vi "subGetBuildSpecificationRefByName.vi"(8 "error in (no error)":errorcluster, 9 "ProjectItem in":refnum<class "ProjectItem.lvclass">, 11 "BuildManager in":refnum<class "BuildManager.lvclass">) -> (0 "error out":errorcluster, 1 "Build spec ref":refnum<vi>, 3 "BuildManager out":refnum<class "BuildManager.lvclass">)   [LabVIEW 2019, in "SolutionBuilder.lvlib" / "BuildManager.lvclass"]
uses:
  BuildManager.lvclass
  ProjectItem/ProjectItem.lvclass
  ProjectItem/ProjectItem.lvclass/ProjectItem.ctl
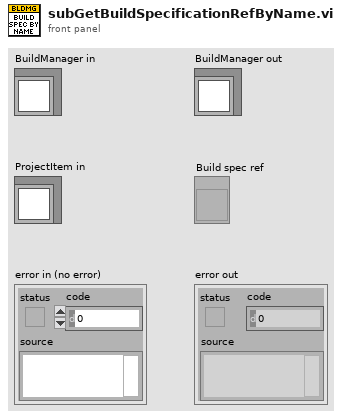
[diagram p1: front panel]
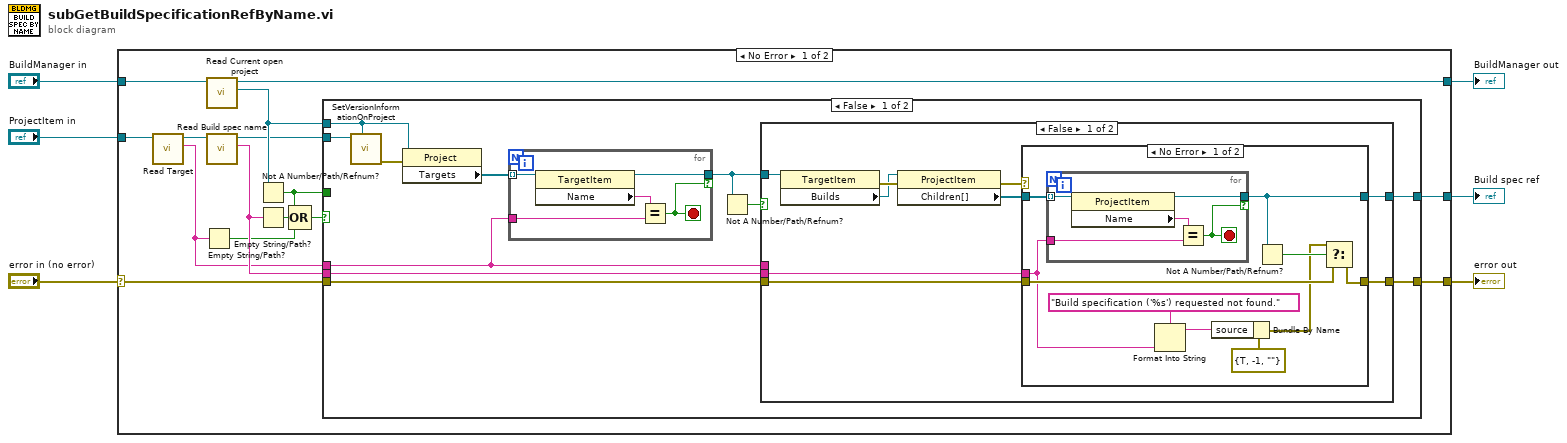
[diagram p0: block diagram]
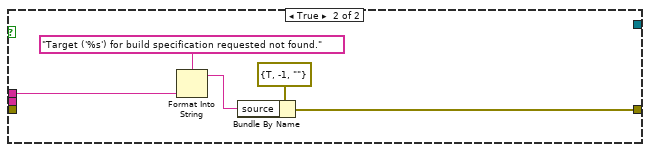
[diagram p3: hidden frame]
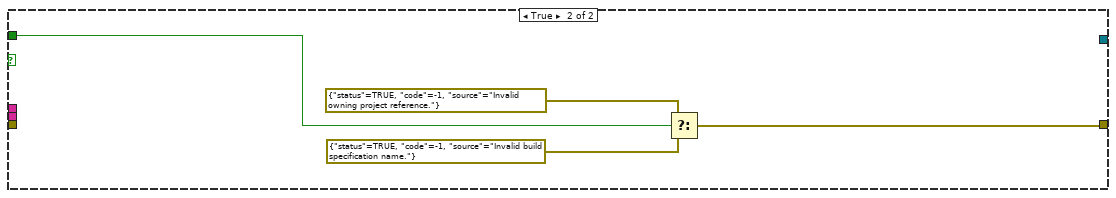
[diagram p4: hidden frame]
diagram:
  n1 = case shown="No Error" "error in (no error)" {
    selector: "error in (no error)" -> [w20 w73]
    tunnel: [w21 _] -> w6
    tunnel: [w19 w73] -> w4
    tunnel: "BuildManager in" -> [w8 w72]
    tunnel: [w15 w72] -> w2
    tunnel: "ProjectItem in" -> [w12 _]
    frame No Error {
      n2 = call "Read Target.vi"("ProjectItem in"=w12) -> ("Target"=w10:string, "ProjectItem out"=w11:refnum<class "ProjectItem.lvclass">)  [unwired: 9 in]
      n3 = Empty String/Path?(string/path=w10) -> (empty?=w9:bool)
      n4 = call "Read Current open project.vi"("BuildManager in"=w8) -> ("Current open project"=w14:refnum<vi>, "BuildManager out"=w15:refnum<class "BuildManager.lvclass">)  [unwired: 9 in]
      n5 = call "Read Build spec name.vi"("ProjectItem in"=w11) -> ("Build spec name"=w13:string, "ProjectItem out"=w7:refnum<class "ProjectItem.lvclass">)  [unwired: 9 in]
      n6 = Not A Number/Path/Refnum?(number/path/refnum=w14) -> (NaN/Path/Refnum?=w16:bool)
      n7 = Empty String/Path?(string/path=w13) -> (empty?=w18:bool)
      n8 = Compound Arithmetic op=OR(w16, w18, w9) -> (w17:bool)
      n9 = case shown="False" w17 {
        tunnel: w13 -> [w32 _]
        tunnel: [w31 _] -> w21
        tunnel: w14 -> [w23 _]
        tunnel: w20 -> [w30 _]
        tunnel: [w29 w69] -> w19
        tunnel: w16 -> [_ w71]
        tunnel: w10 -> [w22 _]
        tunnel: w7 -> [w25 _]
        frame False {
          n10 = call "SetVersionInformationOnProject.vi"("Project ref"=w23, "ProjectItem in"=w25) -> ("error out"=w24:errorcluster)  [unwired: 8 in, 1 out]
          n11 = property class="Project"(reference=w23, error in=w24) -> ("Targets"=w28:refnum<vi>[])  [unwired: 2 out]
          n12 = for {
            tunnel: w28 -> [w67] mode=indexing
            tunnel: w22 -> [w65]
            tunnel: [w64] -> w27 if=w63
            stop <- w63 stop-if-true
            n13 = property class="TargetItem"(reference=w67) -> (reference out=w64:refnum<vi>, "Name"=w66:string)  [unwired: 1 in, 1 out]
            n14 = Equal?(x=w66, y=w65) -> (x = y?=w63:bool)
          }
          n15 = Not A Number/Path/Refnum?(number/path/refnum=w27) -> (NaN/Path/Refnum?=w26:bool)
          n16 = case shown="False" w26 {
            tunnel: w32 -> [w38 _]
            tunnel: [w37 _] -> w31
            tunnel: w30 -> [w35 _]
            tunnel: [w34 w59] -> w29
            tunnel: w27 -> [w33 _]
            tunnel: w22 -> [_ w61]
            frame False {
              n17 = property class="TargetItem"(reference=w33) -> (error out=w41:errorcluster, "Builds"=w39:refnum<vi>)  [unwired: 1 in, 1 out]
              n18 = property class="ProjectItem"(reference=w39, error in=w41) -> (error out=w36:errorcluster, "Children[]"=w40:refnum<vi>[])  [unwired: 1 out]
              n19 = case shown="No Error" w36 {
                selector: w36 -> [_ w57]
                tunnel: w40 -> [w51 _]
                tunnel: w38 -> [w43 _]
                tunnel: [w50 _] -> w37
                tunnel: w35 -> [w48 _]
                tunnel: [w47 w57] -> w34
                frame No Error {
                  n20 = for {
                    tunnel: w51 -> [w56] mode=indexing
                    tunnel: w43 -> [w54]
                    tunnel: [w53] -> w50 if=w52
                    stop <- w52 stop-if-true
                    n21 = property class="ProjectItem"(reference=w56) -> (reference out=w53:refnum<vi>, "Name"=w55:string)  [unwired: 1 in, 1 out]
                    n22 = Equal?(x=w55, y=w54) -> (x = y?=w52:bool)
                  }
                  n23 = Format Into String(format string="Build specification ('%s') requested not found." ("source"), w43) -> (resulting string=w45:string)  [unwired: 2 in, 1 out]
                  n24 = Bundle By Name(cluster=errorcluster {"status"=TRUE, "code"=-1, "source"=""} ("t"), "source"=w45) -> (w44:errorcluster)
                  n25 = Not A Number/Path/Refnum?(number/path/refnum=w50) -> (NaN/Path/Refnum?=w49:bool)
                  n26 = Select(t=w44, s=w49, f=w48) -> (s? t:f=w47:errorcluster)
                }
                frame Error {
                }
              }
            }
            frame True {
              n27 = Format Into String(format string="Target ('%s') for build specification requested not found." ("source"), w61) -> (resulting string=w58:string)  [unwired: 2 in, 1 out]
              n28 = Bundle By Name(cluster=errorcluster {"status"=TRUE, "code"=-1, "source"=""} ("t"), "source"=w58) -> (w59:errorcluster)
            }
          }
        }
        frame True {
          n29 = Select(t=errorcluster {"status"=TRUE, "code"=-1, "source"="Invalid owning project reference."}, s=w71, f=errorcluster {"status"=TRUE, "code"=-1, "source"="Invalid build specification name."} ("t")) -> (s? t:f=w69:errorcluster)
        }
      }
    }
    frame Error {
    }
  }
  "error out" <- w4
  "BuildManager out" <- w2
  "Build spec ref" <- w6
